vi "test31-MappingRelationshipByLocalRegistration_WIthoutSubscriberName_State.vi"(8 "error in (no error)":errorcluster, 11 "TestCase in":refnum<class "testcase-CSMBroadcast.lvclass">) -> (0 "error out":errorcluster, 3 "TestCase out":refnum<class "testcase-CSMBroadcast.lvclass">)   [LabVIEW 2017, in "testcase-CSMBroadcast.lvclass"]
uses:
  testcase-CSMBroadcast.lvclass
  47fe1622-87c8-40c1-b9cf-9bbb5cd90bb5.vi
  <vilib>/addons/_JKI Toolkits/VI Tester/TestCase.llb/TestCase.lvclass
  src/user.lib/_NEVSTOP/Communicable State Machine(CSM)/Communicable State Machine.lvlib
  C:/Program Files (x86)/National Instruments/LabVIEW 2017/vi.lib/addons/_JKI Toolkits/VI Tester/TestCase.llb/TestCase.lvclass
panel:
  out "Loop Count":i32
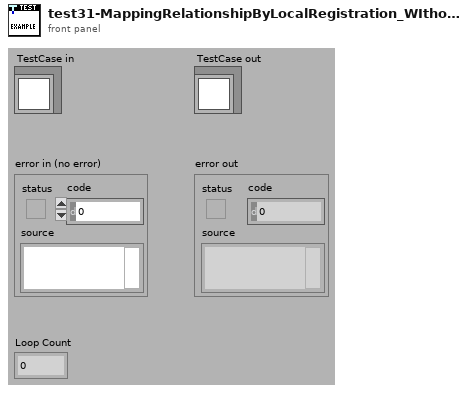
[diagram p1: front panel]
types:
  T1 = cluster{"Status":string, "Source CSM":string, "Target CSM":string, "Target API":string}[]
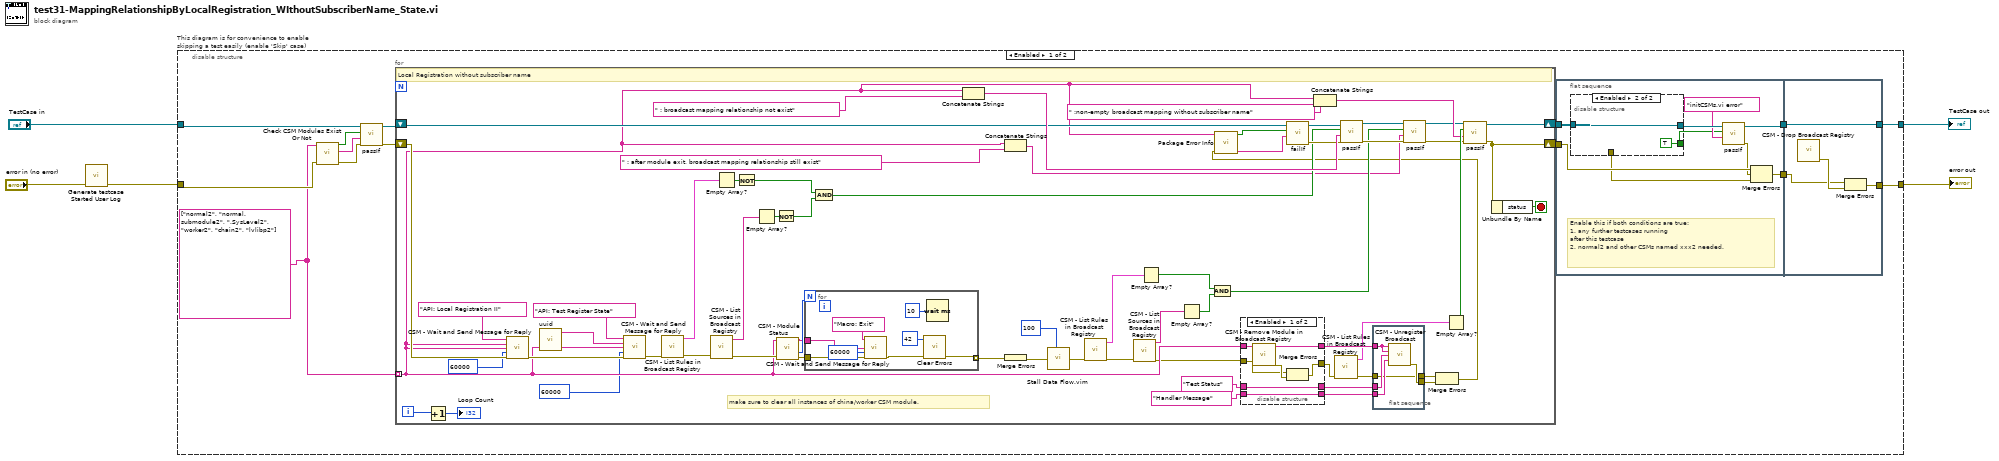
[diagram p0: block diagram]
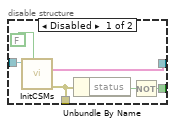
[diagram p2: hidden frame]
diagram:
  n1 = call "Generate testcase Started User Log.vi"("Error In"="error in (no error)") -> ("error out"=w1:errorcluster)  [unwired: 10 in]
  n2 = disable-structure "This diagram is for convenience to enable skipping a test easily (enable 'Skip' case)" shown="Enabled" {
    disable-tunnel: "TestCase in" -> [w16 w132]
    disable-tunnel: [w10 w130] -> w2
    disable-tunnel: [w9 w131] -> w4
    disable-tunnel: w1 -> [w15 w129]
    frame Enabled {
      w6 = string[] ["normal2", "normal.submodule2", ".SysLevel2", "worker2", "chain2", "lvlibp2"]
      n3 = call "Check CSM Modules Exist Or Not.vi"("error in"=w15, "CSM names in"=w6) -> ("error out"=w17:errorcluster, "Debug string"=w18:string, "All Modules Exist?"=w19:bool)  [unwired: 7 in]
      n4 = call-dynamic "passIf.vi"("error in (no error)"=w17, "message (\"\")"=w18, "pass"=w19, "TestCase in"=w16) -> ("error out"=w7:errorcluster, "TestCase out"=w8:refnum<class "testcase-CSMBroadcast.lvclass">)  [unwired: 6 in]
      n5 = for {
        tunnel: w6 -> [w48] mode=indexing
        shift-right: [w88] -> w12
        shift-left: w8 -> [w71]
        shift-right: [w89] -> w11
        shift-left: w7 -> [w86]
        i -> [w95]
        stop <- w98 stop-if-true
        # "make sure to clear all instances of china/worker CSM module."
        # "Local Registration without subscriber name"
        n6 = Increment(x=w95) -> (x+1=→"Loop Count":i32)
        n7 = call "CSM - Wait and Send Message for Reply.vi"("State"="API: Local Registration II", "Arguments (\"\")"=w48, "Target Module"=w48, "Wait (5000ms)"=60000, "Error In (No Error)"=w86) -> ("error out"=w103:errorcluster)  [unwired: 7 in, 3 out]
        n8 = call "uuid.vi"() -> ("UUID"=w101:string)  [unwired: 11 in]
        n9 = call "CSM - Wait and Send Message for Reply.vi"("State"="API: Test Register State", "Arguments (\"\")"=w101, "Target Module"=w48, "Wait (5000ms)"=60000, "Error In (No Error)"=w103) -> ("error out"=w100:errorcluster)  [unwired: 7 in, 3 out]
        n10 = call "CSM - List Rules in Broadcast Registry.vi"("error in (no error)"=w100) -> ("error out"=w97:errorcluster, "Rule Entries"=w93:T1)  [unwired: 8 in, 1 out]
        n11 = call "CSM - List Sources in Broadcast Registry.vi"("error in (no error)"=w97) -> ("error out"=w83:errorcluster, "Broadcast Names"=w90:string[])  [unwired: 9 in]
        n12 = Empty Array?(array=w93) -> (empty?=w92:bool)
        n13 = Not(x=w92) -> (.not. x?=w69:bool)
        n14 = Empty Array?(array=w90) -> (empty?=w91:bool)
        n15 = Not(x=w91) -> (.not. x?=w68:bool)
        n16 = call "CSM - Module Status.vi"("Error In"=w83, "CSM Name"=w48) -> ("error out"=w82:errorcluster, "#Nodes"=w85:i32, "CSM Name (Dup)"=w84:string)  [unwired: 5 in, 2 out]
        n17 = for {
          N: w85 -> [_]
          tunnel: [w123] -> w99 mode=indexing
          tunnel: w84 -> [w127]
          tunnel: w82 -> [w126]
          n18 = call "CSM - Wait and Send Message for Reply.vi"("State"="Macro: Exit", "Target Module"=w127, "Wait (5000ms)"=60000, "Error In (No Error)"=w126) -> ("error out"=w124:errorcluster)  [unwired: 8 in, 3 out]
          n19 = call <vilib>:"Clear Errors.vi"("error in (no error)"=w124, "specific error code to clear (0: all)"=42) -> ("error out"=w123:errorcluster)  [unwired: 4 in, 1 out]
          n20 = Wait (ms)(milliseconds to wait=u32 10) -> ()  [unwired: 1 out]
        }
        n21 = And(x=w69, y=w68) -> (x .and. y?=w67:bool)
        n22 = Concatenate Strings(w48, " : broadcast mapping relationship not exist" ("string")) -> (w78:string)
        n23 = Concatenate Strings(w48, " : after module exit, broadcast mapping relationship still exist" ("string")) -> (w56:string)
        n24 = Merge Errors(w99) -> (w77:errorcluster)
        n25 = call "Stall Data Flow.vim"("value in"=w77, "milliseconds to wait"=u32 100) -> ("value out"=w76:errorcluster)  [unwired: 1 out]
        n26 = call "CSM - List Rules in Broadcast Registry.vi"("error in (no error)"=w76) -> ("error out"=w96:errorcluster, "Rule Entries"=w62:T1)  [unwired: 8 in, 1 out]
        n27 = call "CSM - List Sources in Broadcast Registry.vi"("error in (no error)"=w96) -> ("error out"=w47:errorcluster, "Broadcast Names"=w61:string[])  [unwired: 9 in]
        n28 = Empty Array?(array=w62) -> (empty?=w60:bool)
        n29 = Empty Array?(array=w61) -> (empty?=w59:bool)
        n30 = And(x=w60, y=w59) -> (x .and. y?=w58:bool)
        n31 = disable-structure shown="Enabled" {
          disable-tunnel: w47 -> [w110 w119]
          disable-tunnel: [w114 w119] -> w54
          disable-tunnel: w48 -> [w115 w120]
          disable-tunnel: "Test Status" ("Status") -> [w112 w118]
          disable-tunnel: "Handler Message" ("Response Message (If \"\", Same as Source Message)") -> [w111 w117]
          disable-tunnel: [w113 w120] -> w55
          disable-tunnel: [w112 w118] -> w53
          disable-tunnel: [w111 w117] -> w52
          frame Enabled {
            n32 = call "CSM - Remove Module in Broadcast Registry.vi"("CSM Name"=w115) -> ("CSM Name (Dup)"=w113:string, "error out"=w116:errorcluster)  [unwired: 13 in]
            n33 = Merge Errors(w110, w116) -> (w114:errorcluster)
          }
          frame Disabled {
          }
        }
        n34 = Concatenate Strings(w48, " :non-empty broadcast mapping without subscriber name" ("string")) -> (w79:string)
        n35 = call "CSM - List Rules in Broadcast Registry.vi"("error in (no error)"=w54) -> ("error out"=w50:errorcluster, "Rule Entries"=w43:T1)  [unwired: 8 in, 1 out]
        n36 = flat-sequence {
          tunnel: w55 -> [w109]
          tunnel: w53 -> [w108]
          tunnel: w52 -> [w107]
          tunnel: [w106] -> w51
          tunnel: w50 -> [w105]
          tunnel: [w105] -> w49
          frame #0 {
            n37 = call "CSM - Unregister Broadcast.vi"("CSM Name(Empty for Broadcast Event)"=w109, "Source CSM Name (* as Default)"=w109, "Trigger"=w108, "API (\"*\" as Default)"=w107) -> ("error out"=w106:errorcluster)  [unwired: 10 in, 1 out]
          }
        }
        n38 = Merge Errors(w49, w51) -> (w46:errorcluster)
        n39 = call "Package Error Info.vi"("error in"=w46, "String in"=w48) -> ("packed error info out"=w74:string, "error status"=w73:bool)  [unwired: 8 in]
        n40 = call-dynamic "failIf.vi"("message (\"\")"=w74, "fail"=w73, "TestCase in"=w71) -> ("error out"=w72:errorcluster, "TestCase out"=w70:refnum<class "testcase-CSMBroadcast.lvclass">)  [unwired: 7 in]
        n41 = call-dynamic "passIf.vi"("error in (no error)"=w72, "message (\"\")"=w78, "pass"=w67, "TestCase in"=w70) -> ("error out"=w64:errorcluster, "TestCase out"=w66:refnum<class "testcase-CSMBroadcast.lvclass">)  [unwired: 6 in]
        n42 = call-dynamic "passIf.vi"("error in (no error)"=w64, "message (\"\")"=w56, "pass"=w58, "TestCase in"=w66) -> ("error out"=w63:errorcluster, "TestCase out"=w65:refnum<class "testcase-CSMBroadcast.lvclass">)  [unwired: 6 in]
        n43 = Empty Array?(array=w43) -> (empty?=w87:bool)
        n44 = call-dynamic "passIf.vi"("error in (no error)"=w63, "message (\"\")"=w79, "pass"=w87, "TestCase in"=w65) -> ("error out"=w89:errorcluster, "TestCase out"=w88:refnum<class "testcase-CSMBroadcast.lvclass">)  [unwired: 6 in]
        n45 = Unbundle By Name(w89) -> ("status"=w98:bool)
      }
      n46 = flat-sequence {
        tunnel: w12 -> [w28]
        tunnel: [w26] -> w14
        tunnel: w11 -> [w24]
        tunnel: [w21] -> w13
        tunnel: w14 -> [w39]
        tunnel: [w39] -> w10
        tunnel: [w38] -> w9
        tunnel: w13 -> [w37]
        frame #0 {
          # "Enable this if both conditions are true:\n1. any further testcases running\nafter this testcase\n2. normal2 and other CSMs named xxx2 needed."
          n47 = disable-structure shown="Enabled" {
            disable-tunnel: w28 -> [w34 w36]
            disable-tunnel: [w32 w36] -> w27
            disable-tunnel: [w30 _] -> w22
            disable-tunnel: [w29 TRUE ("pass")] -> w20
            frame Disabled {
              n48 = call "InitCSMs.vi"(7:FALSE ("Enable building lvlibp?"), 11:w34) -> ("error out"=w30:errorcluster, "CSMs"=w32:string[])  [unwired: 8 in]
              n49 = Unbundle By Name(w30) -> ("status"=w31:bool)
              n50 = Not(x=w31) -> (.not. x?=w29:bool)
            }
            frame Enabled {
            }
          }
          n51 = call-dynamic "passIf.vi"("message (\"\")"="initCSMs.vi error" ("message (\"\")"), "pass"=w20, "TestCase in"=w27) -> ("error out"=w23:errorcluster, "TestCase out"=w26:refnum<class "testcase-CSMBroadcast.lvclass">)  [unwired: 7 in]
          n52 = Merge Errors(w24, w23, w22) -> (w21:errorcluster)
        }
        frame #1 {
          n53 = call "CSM - Drop Broadcast Registry.vi"() -> ("error out"=w40:errorcluster)  [unwired: 15 in]
          n54 = Merge Errors(w37, w40) -> (w38:errorcluster)
        }
      }
    }
    frame Disabled {
      # "skip test result while test is under development"
      n55 = call <vilib>:"skip.vi"("error in (no error)"=w129, "TestCase in"=w132) -> ("error out"=w131:errorcluster, "TestCase out"=w130:refnum<class "testcase-CSMBroadcast.lvclass">)  [unwired: 8 in]
    }
  }
  "error out" <- w4
  "TestCase out" <- w2
